vi "DAC Init Results.vi"(8 "error in":errorcluster, 9 "Log Details?":bool, 10 "tdms file":refnum<k34>, 11 "DAC Vacum Pressure in":refnum<class "DAC Vacum Pressure.lvclass">) -> (0 "error out":errorcluster, 2 "tdms file out":refnum<k34>)   [LabVIEW 2019, in "DAC.lvlib" / "DAC Vacum Pressure.lvclass"]
uses:
  DAC Vacum Pressure.lvclass
  DAC.lvclass
  C:/Users/wg/Documents/LV_Projects/test-stand/App/DAC/DAC.lvclass
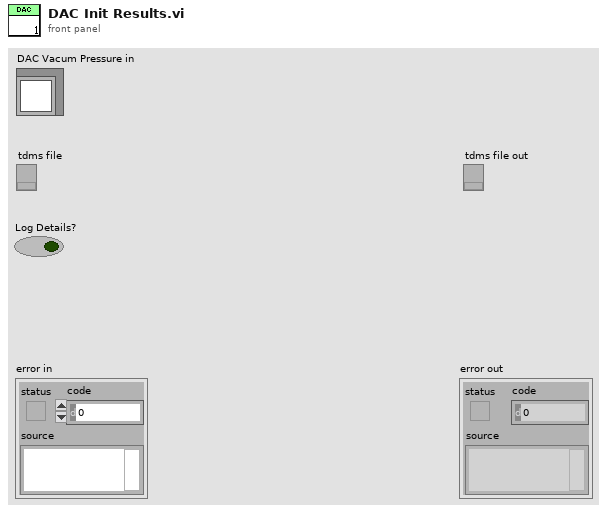
[diagram p1: front panel]
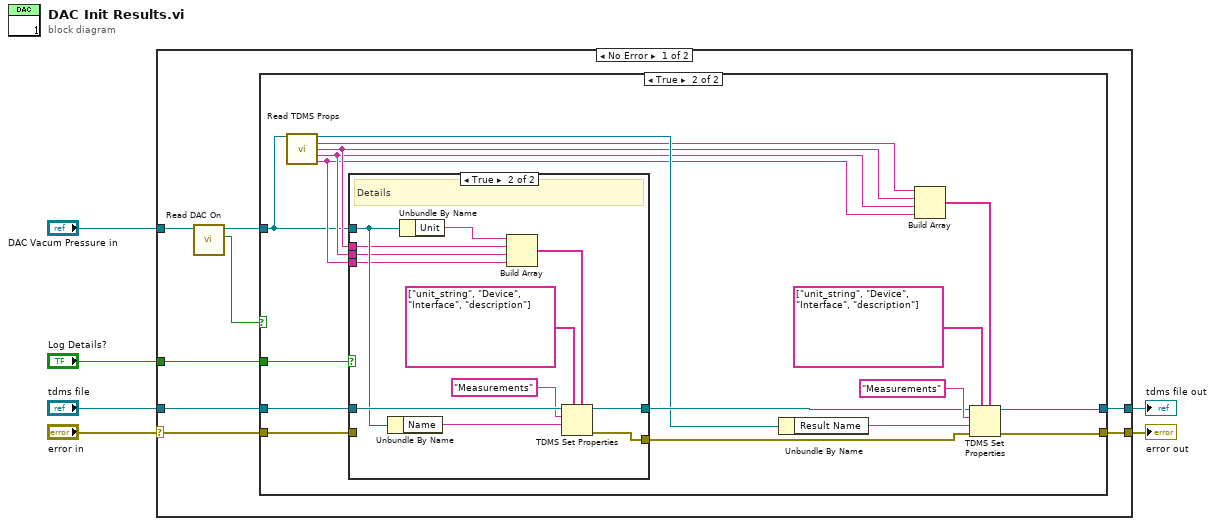
[diagram p0: block diagram]
diagram:
  n1 = case shown="No Error" "error in" {
    selector: "error in" -> [w10 w49]
    tunnel: [w7 w49] -> w6
    tunnel: "DAC Vacum Pressure in" -> [w14 _]
    tunnel: "tdms file" -> [w11 w48]
    tunnel: [w8 w48] -> w5
    tunnel: "Log Details?" -> [w9 _]
    frame No Error {
      n2 = call "Read DAC On.vi"("DAC in"=w14) -> ("DAC On"=w12:bool, "DAC out"=w13:refnum<class "DAC Vacum Pressure.lvclass">)  [unwired: 8 in, 1 out]
      n3 = case shown="True" w12 {
        tunnel: w11 -> [w15 w20]
        tunnel: [w15 w18] -> w8
        tunnel: [w16 w17] -> w7
        tunnel: w13 -> [_ w21]
        tunnel: w10 -> [w16 w19]
        tunnel: w9 -> [_ w22]
        frame False {
        }
        frame True {
          n4 = call "Read TDMS Props.vi"("DAC in"=w21) -> ("DAC out"=w28:refnum<class "DAC Vacum Pressure.lvclass">, "Result Unit"=w26:string, "DAC Device"=w25:string, "DAC IO"=w24:string, "DAC Description"=w23:string)  [unwired: 10 in]
          n5 = case shown="True" w22 {
            tunnel: w20 -> [w35 w47]
            tunnel: [w35 w43] -> w30
            tunnel: [w34 w42] -> w29
            tunnel: w21 -> [_ w40]
            tunnel: w19 -> [w34 _]
            tunnel: w25 -> [_ w38]
            tunnel: w24 -> [_ w37]
            tunnel: w23 -> [_ w36]
            frame False {
            }
            frame True {
              # "Details"
              n6 = Unbundle By Name(w40) -> ("Name"=w41:string)
              n7 = Unbundle By Name(w40) -> ("Unit"=w45:string)
              n8 = Build Array(w45, w38, w37, w36) -> (w44:string[])
              n9 = TDMS Set Properties(5:w44, 7:string[] ["unit_string", "Device", "Interface", "description"] ("property names"), 9:w41, 10:"Measurements" ("group name in (Untitled)"), 11:w47) -> (0:w42:errorcluster, 3:w43:refnum<k34>)  [unwired: 1 in, 2 out]
            }
          }
          n10 = Unbundle By Name(w28) -> ("Result Name"=w31:string)
          n11 = Build Array(w26, w25, w24, w23) -> (w32:string[])
          n12 = TDMS Set Properties(5:w32, 7:string[] ["unit_string", "Device", "Interface", "description"] ("property names"), 8:w29, 9:w31, 10:"Measurements" ("group name in (Untitled)"), 11:w30) -> (0:w17:errorcluster, 3:w18:refnum<k34>)  [unwired: 2 out]
        }
      }
    }
    frame Error {
    }
  }
  "error out" <- w6
  "tdms file out" <- w5
